vi "Prime BSI Camera Engine.vi"(0 "Notifier Name":string, 11 "Camera Index and Px Size":string[](array[string])) -> ()   [LabVIEW 2018]
uses:
  Z:/Software/Photometrics/Photometrics LabView Package 2021/Dependencies/PVCamNET.dll
  IDS/IDS Controls/IDS ROI.ctl
  <vilib>/vision/Image Controls.llb/IMAQ Image.ctl
  Prime BSI Type Defs/Prime BSI Notifier Element.ctl
  Prime BSI Type Defs/Prime BSI Parameter List.ctl
  Prime BSI Type Defs/Prime BSI Parameters.ctl
  Prime BSI Type Defs/Prime BSI Actions.ctl
  shell32.dll
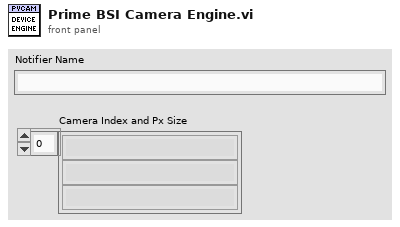
[diagram p1: front panel]
types:
  T1 = typedef "Prime BSI Actions.ctl" = enum16{"Do Nothing", "Initialize", "Preview", "Record", "Abort", "Record Settings", "Set Parameter", "Get Parameter", "Set ROI", "Get ROI", "Status", "Quit"}
  T2 = typedef "Prime BSI Notifier Element.ctl" = cluster{"PVCam Actions":T1, "Received?":bool, "PVCam Parameter":T3, "PVCam ROI":T5, "Running?":bool, "File Path":path, "# of frames":u32, "Image Ref":T6, "Binning":i32}
  T3 = typedef "Prime BSI Parameters.ctl" = cluster{"Parameter":T4, "Value":dbl}
  T4 = typedef "Prime BSI Parameter List.ctl" = enum16{"Exposure Time (s)", "Binning"}
  T5 = typedef "IDS ROI.ctl" = cluster{"H Offset":i32, "V Offset":i32, "H Width":i32, "V Width":i32}
  T6 = typedef "IMAQ Image.ctl" = refnum<image>
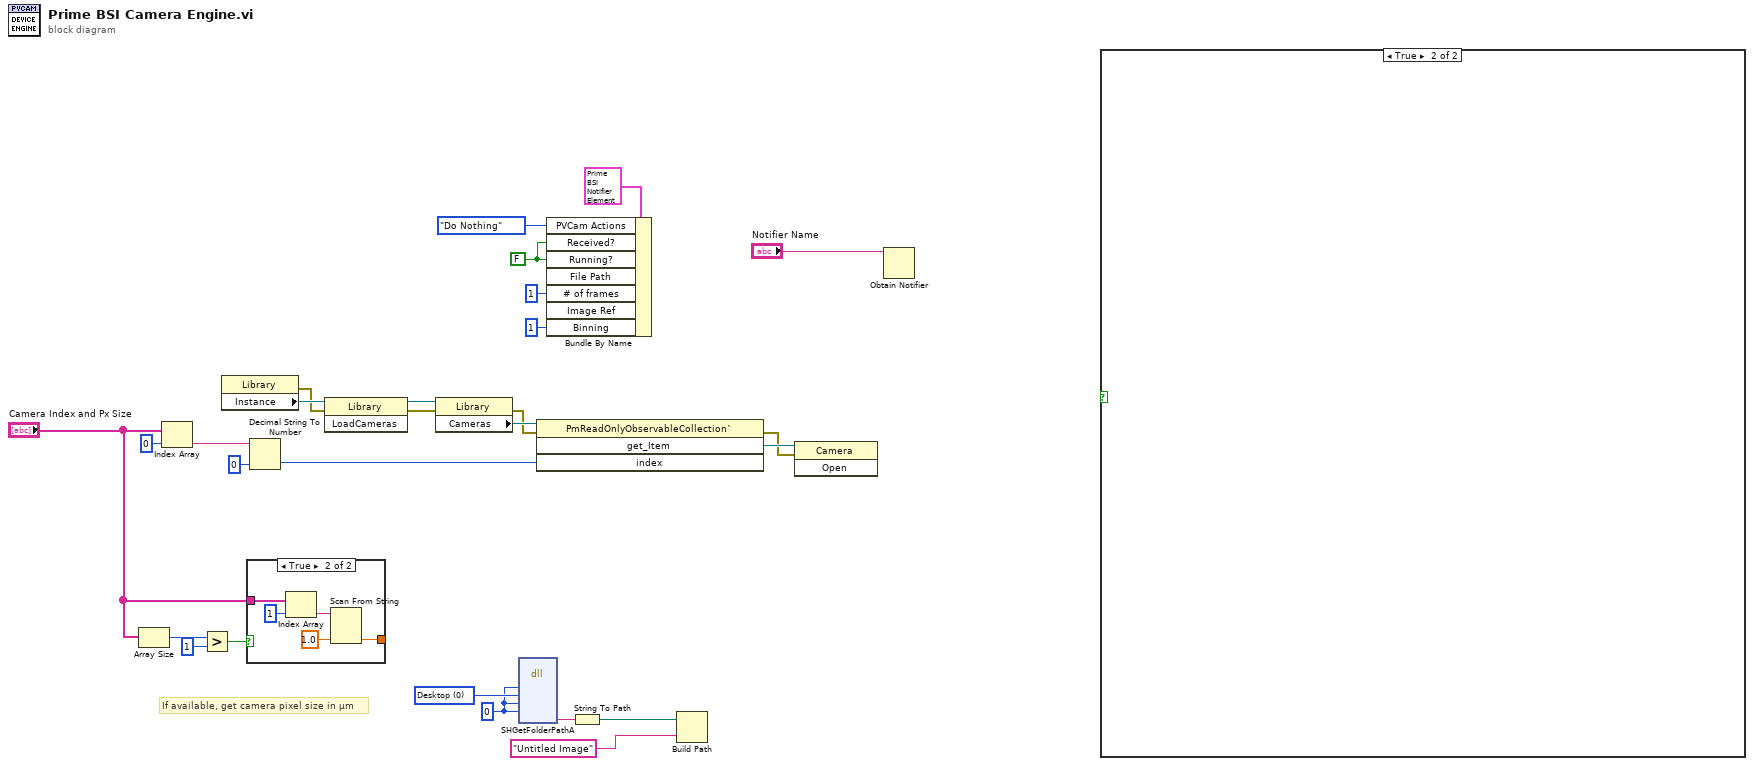
[diagram p0: block diagram]
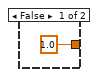
[diagram p3: hidden frame]
diagram:
  w5 = 0 items=["Desktop"=0, "Personal Documents"=5, "AppData"=26, "Local AppData"=28, "Common AppData"=35, "Program Files"=38, "Program Files Common"=43, "Common Documents"=46] ("Requested Path")
  w4 = 0 ("HWND")
  w6 = FALSE ("Running?")
  # "If available, get camera pixel size in µm"
  n1 = Array Size(array="Camera Index and Px Size") -> (size(s)=w22:i32)
  n2 = Index Array(array="Camera Index and Px Size", index=0) -> (element=w23:string)
  n3 = Greater?(x=w22, y=1) -> (0:w21:bool)
  n4 = property class="Library"() -> (error out=w17:errorcluster, "Instance"=w27:refnum<k24>)  [unwired: 2 in, 1 out]
  n5 = case shown="True" w21 {
    tunnel: "Camera Index and Px Size" -> [_ w31]
    tunnel: [1.0 ("default (0 dbl)") w33] -> _
    frame False {
    }
    frame True {
      n6 = Index Array(array=w31, index=1) -> (element=w32:string)
      n7 = Scan From String(input string=w32, default 1=1.0 ("default (0 dbl)")) -> (output 1=w33:dbl)  [unwired: 3 in, 3 out]
    }
  }
  n8 = Decimal String To Number(string=w23, default (0L)=0 ("default (0 I32)")) -> (number=w14:i32)  [unwired: 1 in, 1 out]
  n9 = invoke class="Library" method="LoadCameras"(reference=w27, error in=w17) -> (reference out=w26:refnum<k24>, error out=w16:errorcluster)  [unwired: 1 in, 1 out]
  n10 = property class="Library"(reference=w26, error in=w16) -> (error out=w15:errorcluster, "Cameras"=w18:refnum<k24>)  [unwired: 1 out]
  n11 = dll-call lib="shell32.dll" fn="SHGetFolderPathA"("HWND"=w4, "nFolder"=w5, "hToken"=w4, "dwFlags"=w4) -> ("pszPath"=w3:string)  [unwired: 9 in, 2 out]
  n12 = invoke class="PmReadOnlyObservableCollection`" method="get_Item"(reference=w18, error in=w15, "index"=w14) -> (error out=w12:errorcluster, "get_Item"=w13:refnum<k24>)  [unwired: 1 in, 2 out]
  n13 = Bundle By Name(cluster=T2 {"PVCam Actions"=enum."Do Nothing", "Received?"=FALSE, "PVCam Parameter"={"Parameter"=enum."Exposure Time (s)", "Value"=0.0}, "PVCam ROI"={"H Offset"=0, "V Offset"=0, "H Width"=0, "V Width"=0}, "Running?"=FALSE, "File Path"=path "", "# of frames"=0, "Image Ref"=refnum, "Binning"=0} ("IDS Camera Cluster"), "PVCam Actions"=Prime_BSI_Actions."Do Nothing", "Received?"=w6, "Running?"=w6, "# of frames"=u32 1, "Binning"=1) -> ()  [unwired: 2 in, 1 out]
  n14 = String To Path(string=w3) -> (path=w1:path)
  n15 = Build Path(base path=w1, name or relative path="Untitled Image") -> ()  [unwired: 1 out]
  n16 = invoke class="Camera" method="Open"(reference=w13, error in=w12) -> ()  [unwired: 1 in, 3 out]
  n17 = Obtain Notifier(name (unnamed)="Notifier Name") -> ()  [unwired: 3 in, 3 out]
  n18 = case shown="True" {
    selector: _ -> [_ _]
    frame False {
    }
    frame True {
    }
  }
